vi "Left Click.vi"(7 "object refs":T2, 8 "error in":errorcluster, 9 "Coords":T1, 10 "Event data":variant, 11 "Multi Column Listbox in":refnum<class "Multi Column Listbox.lvclass">) -> (0 "error out":errorcluster, 2 "Discard?":bool, 3 "Multi Column Listbox out":refnum<class "Multi Column Listbox.lvclass">)   [LabVIEW 2014, in "Table Manager.lvlib" / "Multi Column Listbox.lvclass"]
uses:
  Multi Column Listbox.lvclass
  Table Manager/object ref.ctl
  Configuration Editor/Classes/Engine Parent/Engine Parent Editor Node.lvclass
  Configuration Editor/Classes/Module editor node/module editor node.lvclass
  <vilib>/Utility/miscctls.llb/LVPoint32TypeDef.ctl
  Multi Column Listbox.lvclass/Multi Column Listbox.ctl
  Table Manager/Table Manager.lvclass/Table Manager.ctl
  Line/Line.lvclass/Line.ctl
  Column/Column.lvclass/Column.ctl
  Line/Read Columns.vi
  Line/Write Columns.vi
  Read Listbox.vi
  Table Manager/Read Line.vi
  Table Manager/Read Top VI.vi
  Table Manager/Write Line.vi
  Line/Line.lvclass
  Column/Column.lvclass
  Table Manager/Table Manager.lvclass
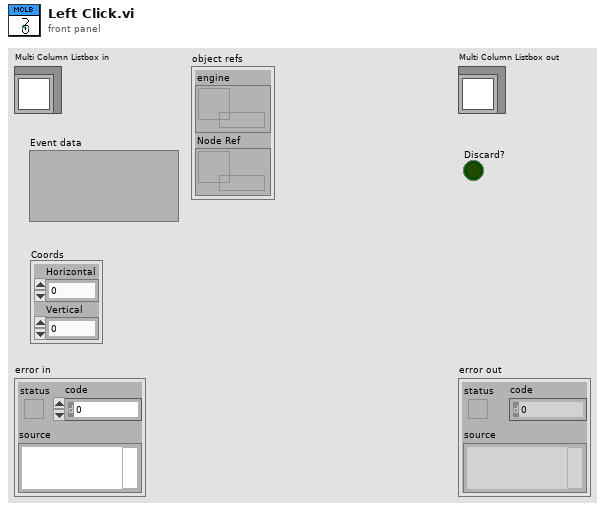
[diagram p1: front panel]
types:
  T1 = typedef "LVPoint32TypeDef.ctl" = cluster{"Horizontal":i32, "Vertical":i32}
  T2 = typedef "Table Manager.lvlib/Table Manager.lvclass/object ref.ctl" = cluster{"engine":refnum<data-value>, "Node Ref":refnum<data-value>}
  T3 = typedef "LVRowAndColumnTypeDef.ctl" = cluster{"Row":i32, "Column":i32}
  T4 = typedef "LVPositionTypeDef.ctl" = cluster{"Left":i32, "Top":i32}
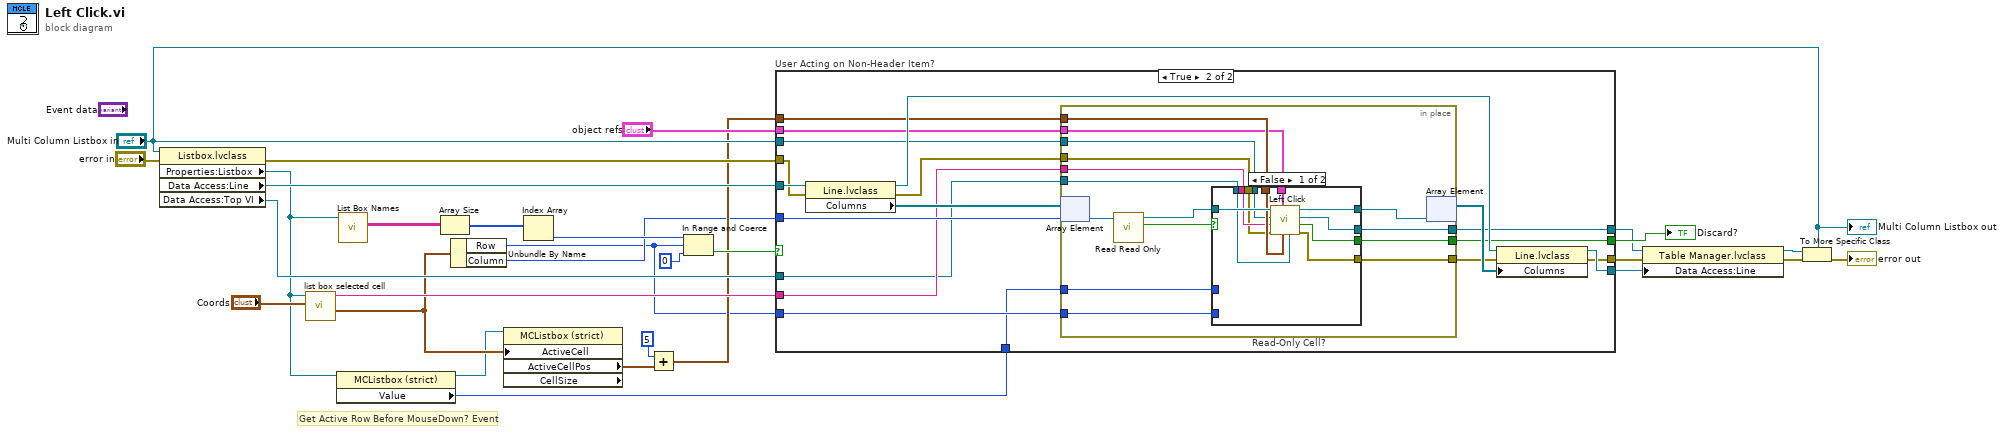
[diagram p0: block diagram]
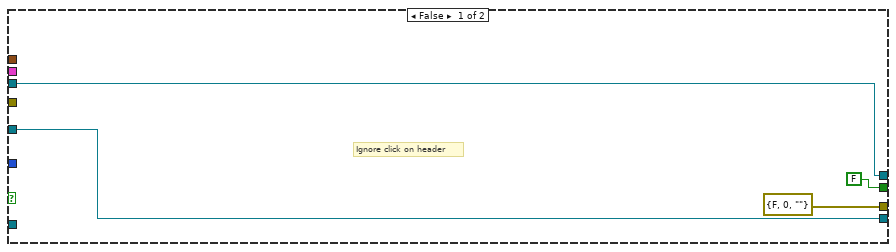
[diagram p2: hidden frame]
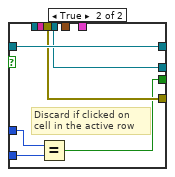
[diagram p3: hidden frame]
diagram:
  # "Get Active Row Before MouseDown? Event"
  n1 = property class="Listbox.lvclass"(reference="Multi Column Listbox in", error in="error in") -> (error out=w13:errorcluster, "Properties:Listbox"=w4:refnum<vi>, "Data Access:Line"=w29:refnum<class "Line.lvclass">, "Data Access:Top VI"=w11:refnum<vi>)  [unwired: 1 out]
  n2 = call "list box selected cell.vi"("Coords"="Coords", "MulticolumnListbox in"=w4) -> ("cell position"=w9:T3, "tag select name"=w20:string)  [unwired: 6 in, 2 out]
  n3 = property class="MCListbox (strict)"(reference=w4) -> (reference out=w3:refnum<vi>, "Value"=w2:i32)  [unwired: 1 in, 1 out]
  n4 = call "List Box Names.vi"("MulticolumnListbox in"=w4) -> ("ItemNames"=w26:string[][])  [unwired: 8 in, 2 out]
  n5 = Array Size(array=w26) -> (size(s)=w25:i32[])
  n6 = Unbundle By Name(w9) -> ("Row"=w1:i32, "Column"=w5:i32)
  n7 = property class="MCListbox (strict)" props=["ActiveCell", "ActiveCellPos", "CellSize"](reference=w3, "ActiveCell"=w9) -> ("ActiveCellPos"=w8:T4)  [unwired: 1 in, 3 out]
  n8 = Index Array(array=w25) -> (element=w24:i32)  [unwired: 1 in]
  n9 = Add(x=5, y=w8) -> (x+y=w6:T4)
  n10 = In Range and Coerce(upper limit=w24, x=w1, lower limit=0) -> (In Range?=w28:bool)  [unwired: 1 out]
  n11 = case "User Acting on Non-Header Item?" shown="True" w28 {
    tunnel: w29 -> [w33 w52]
    tunnel: w5 -> [_ w51]
    tunnel: [w33 w47] -> w23
    tunnel: [errorcluster {"status"=FALSE, "code"=0, "source"=""} ("error out") w46] -> w22
    tunnel: [FALSE ("Discard") w45] -> w21
    tunnel: w6 -> [_ w44]
    tunnel: w20 -> [_ w43]
    tunnel: "Multi Column Listbox in" -> [w30 w42]
    tunnel: [w30 w41] -> w19
    tunnel: "object refs" -> [_ w40]
    tunnel: w13 -> [_ w37]
    tunnel: w11 -> [_ w36]
    tunnel: w2 -> [_ w34]
    tunnel: w1 -> [_ w35]
    frame False {
      # "Ignore click on header"
    }
    frame True {
      n12 = property class="Line.lvclass"(reference=w52, error in=w37) -> (reference out=w48:refnum<class "Line.lvclass">, error out=w39:errorcluster, "Columns"=w50:refnum<class "Column.lvclass">[])
      n13 = in-place {
        in-place-border: [w66] -> w45
        in-place-border: w44 -> [w65]
        in-place-border: w36 -> [w64]
        in-place-border: w43 -> [w63]
        in-place-border: w42 -> [w62]
        in-place-border: [w61] -> w41
        in-place-border: w40 -> [w60]
        in-place-border: w39 -> [w59]
        in-place-border: [w58] -> w38
        in-place-border: w35 -> [w53]
        in-place-border: w34 -> [w54]
        n14 = in-place-array #1(w50, w51) -> (w57:refnum<class "Column.lvclass">)
        n15 = call "Read Read Only.vi"("Column in"=w57) -> ("Read Only"=w55:bool, "Column out"=w56:refnum<class "Column.lvclass">)  [unwired: 8 in, 1 out]
        n16 = case "Read-Only Cell?" shown="False" w55 {
          tunnel: w56 -> [w78 w84]
          tunnel: [w77 w84] -> w67
          tunnel: [w76 w79] -> w66
          tunnel: w65 -> [w75 _]
          tunnel: w64 -> [w74 _]
          tunnel: w63 -> [w73 _]
          tunnel: w62 -> [w72 w83]
          tunnel: [w71 w83] -> w61
          tunnel: w60 -> [w70 _]
          tunnel: w59 -> [w69 w82]
          tunnel: [w68 w82] -> w58
          tunnel: w54 -> [_ w81]
          tunnel: w53 -> [_ w80]
          frame False {
            n17 = call-dynamic "Left Click.vi"("Top  VI"=w74, "Coords"=w75, "object refs"=w70, "error in (no error)"=w69, "line name"=w73, "Table Manager in"=w72, "column in"=w78) -> ("error out"=w68:errorcluster, "Discard"=w76:bool, "Table Manager out"=w71:refnum<class "Table Manager.lvclass">, "column out"=w77:refnum<class "Column.lvclass">)  [unwired: 1 in]
          }
          frame True {
            # "Discard if clicked on cell in the active row"
            n18 = Equal?(x=w81, y=w80) -> (x = y?=w79:bool)
          }
        }
        n19 = in-place-array #1(w67) -> (w49:refnum<class "Column.lvclass">[])  [unwired: 1 out]
      }
      n20 = property class="Line.lvclass"(reference=w48, error in=w38, "Columns"=w49) -> (reference out=w47:refnum<class "Line.lvclass">, error out=w46:errorcluster)
    }
  }
  "Discard?" <- w21
  n21 = property class="Table Manager.lvclass"(reference=w19, error in=w22, "Data Access:Line"=w23) -> (reference out=w17:refnum<class "Table Manager.lvclass">, error out=w16:errorcluster)
  n22 = To More Specific Class(target class="Multi Column Listbox in", reference=w17, error in=w16) -> (error out=→"error out":errorcluster)  [unwired: 1 out]
  "Multi Column Listbox out" <- "Multi Column Listbox in"
